vi "VIH Project Tree - Can Items Be Built.vi"(8 "error in":errorcluster, 9 "Stop when first found (T)":bool=TRUE, 10 "Parent Item Tag (Root)":string, 11 "Project Tree":T1) -> (0 "error out":errorcluster, 1 "with descendants":bool, 2 "Can be built":bool, 3 "dup Project Tree":T1)   [LabVIEW 2014]
doc: "::: VI Helpeks :::\nCopyright (c) 2000-2026 Konstantin Shifershteyn. All rights reserved."
uses:
  VIH Project Tree Typedef - Tree Refnum.ctl
panel:
  # "VI Helpeks\nCopyright (c) 2012-2026 Konstantin Shifershteyn"
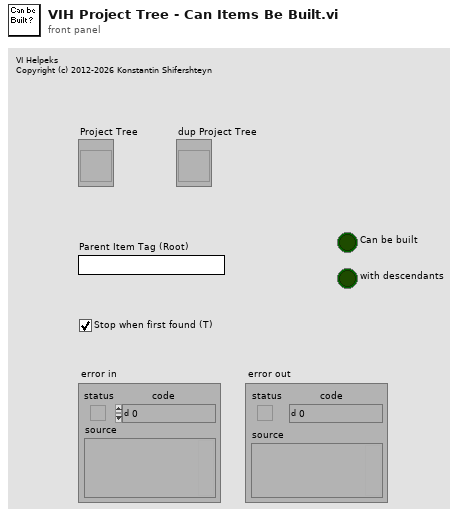
[diagram p1: front panel]
types:
  T1 = typedef "VIH Project Tree Typedef - Tree Refnum.ctl" = refnum<vi>
  T2 = typedef "VIH Project Tree Typedef - Tree Item Type.ctl" = enum32{"<Invalid>", "Project", "Proj Files", "Proj Rules", "File Group", "Rule Group", "Any File", "LV Func", ".mnu", ".mnu (dyn)", ".vi", ".vi (dyn)", ".vit", ".vit (dyn)", ".ctl", ".ctl (dyn)", ".ctt", ".ctt (dyn)", "polyVI", "polyVI (dyn)", "expVI", "expVI (dyn)", "HTML", "PolyVI Inst"}
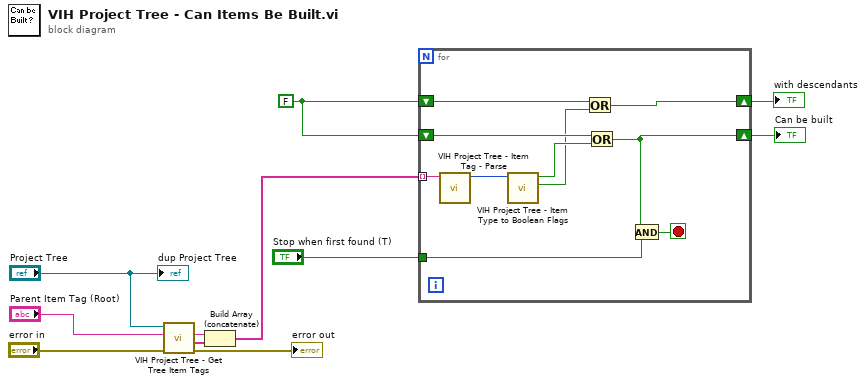
[diagram p0: block diagram]
diagram:
  w4 = FALSE
  n1 = call "VIH Project Tree - Get Tree Item Tags.vi"("error in"="error in", "Parent Item Tag"="Parent Item Tag (Root)", "Project Tree"="Project Tree") -> ("error out"=→"error out":errorcluster, "Child Item Tags"=w7:string[], "dup Parent Item Tag"=w6:string)  [unwired: 5 in, 1 out]
  n2 = Build Array (concatenate)(w6, w7) -> (w5:string[])
  n3 = for {
    tunnel: w5 -> [w21] mode=indexing
    shift-right: [w14] -> w3
    shift-left: w4 -> [w17]
    shift-right: [w12] -> w2
    shift-left: w4 -> [w16]
    tunnel: "Stop when first found (T)" -> [w20]
    stop <- w19 stop-if-true
    n4 = call "VIH Project Tree - Item Tag - Parse.vi"("Tree Item Tag"=w21) -> ("Item Type"=w18:T2)  [unwired: 8 in, 2 out]
    n5 = call "VIH Project Tree - Item Type to Boolean Flags.vi"("Item Type"=w18) -> ("Palette menu"=w13:bool, "Can be built"=w15:bool)  [unwired: 4 in, 5 out]
    n6 = Or(x=w16, y=w13) -> (x .or. y?=w12:bool)
    n7 = Or(x=w17, y=w15) -> (x .or. y?=w14:bool)
    n8 = And(x=w14, y=w20) -> (x .and. y?=w19:bool)
  }
  "with descendants" <- w2
  "Can be built" <- w3
  "dup Project Tree" <- "Project Tree"
